vi "FuncVI-QueueTest.vi"(5 "InstanceRef":T2, 9 "arg list":T1[](array[typedef]) {"num" format="%.2f"}) -> (0 "error out":bool, 3 "result":T1 {"num" format="%.2f"})   [LabVIEW 2021]
doc: "::: CalcExpress Toolkit :::\nCopyright (c) 2000-2026 Konstantin Shifershteyn. All rights reserved."
uses:
  cetypes.llb/CalcExpress Function Argument Info.ctl
  cetypes.llb/CalcExpress Instance RefNum.ctl
panel:
  in  "max arg num":i32=1
  in  "min arg num":i32=1
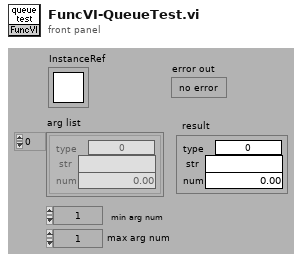
[diagram p1: front panel]
types:
  T1 = typedef "CalcExpress Function Argument Info.ctl" = cluster{"type":u32, "str":string, "num":dbl}
  T2 = typedef "CalcExpress Instance RefNum.ctl" = refnum<k1>
  T3 = enum32{"String", "DBL Number", "identifier", "1D Array of DBL", "2D Array of DBL", "CDB Number", "1D Array of CDB", "2D Array of CDB", "1D Array of String", "2D Array of String", "Unknown data type"}
  T4 = cluster{"data type":enum32{"String", "DBL Number", "identifier", "1D Array of DBL", "2D Array of DBL", "CDB Number", "1D Array of CDB", "2D Array of CDB", "1D Array of String", "2D Array of String", "Unknown data type"}, string, dbl}
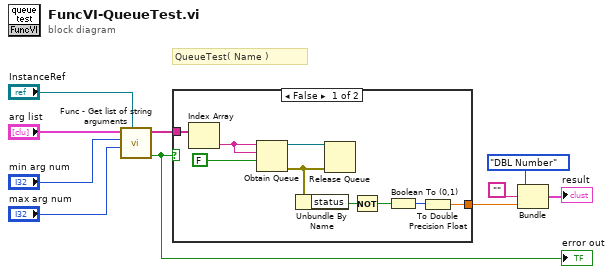
[diagram p0: block diagram]
diagram:
  # "QueueTest( Name )"
  n1 = call "Func - Get list of string arguments.vi"("InstanceRef"="InstanceRef", "max arg num"="max arg num", "min arg num"="min arg num", "arg list"="arg list") -> ("error out"=w8:bool, "val list"=w9:string[])  [unwired: 4 in]
  "error out" <- w8
  n2 = case shown="False" w8 {
    tunnel: w9 -> [w19 _]
    tunnel: [w11 _] -> w1
    frame False {
      n3 = Index Array(array=w19) -> (element=w17:string)  [unwired: 1 in]
      n4 = Obtain Queue(name (unnamed)=w17, element data type=w17, create if not found? (T)=FALSE) -> (queue out=w15:refnum<queue>, error out=w14:errorcluster)  [unwired: 2 in, 1 out]
      n5 = Unbundle By Name(w14) -> ("status"=w18:bool)
      n6 = Release Queue(queue=w15, error in (no error)=w14) -> ()  [unwired: 1 in, 3 out]
      n7 = Not(x=w18) -> (.not. x?=w13:bool)
      n8 = Boolean To (0,1)(Boolean=w13) -> (0, 1=w12:i16)
      n9 = To Double Precision Float(number=w12) -> (double precision float=w11:dbl)
    }
    frame True {
    }
  }
  n10 = Bundle("data type"=T3."DBL Number", "", w1) -> (→"result":T4)  [unwired: 1 in]
